vi "Set Input.vi"(8 "error in (no error)":errorcluster caption="에러 입력(에러 없음)", 10 "Input path":T1, 11 "CE RF Switch Box 입력":refnum<class "CE RF Switch Box.lvclass">) -> (0 "error out":errorcluster caption="에러 출력", 3 "CE RF Switch Box 출력":refnum<class "CE RF Switch Box.lvclass">)   [LabVIEW 2023, in "RF Switch Box.lvlib" / "CE RF Switch Box.lvclass"]
uses:
  CE RF Switch Box.lvclass
  Type Definition/Input path.ctl
  CE RF Switch Box.lvclass/CE RF Switch Box.ctl
  RF Switch Box.lvlib
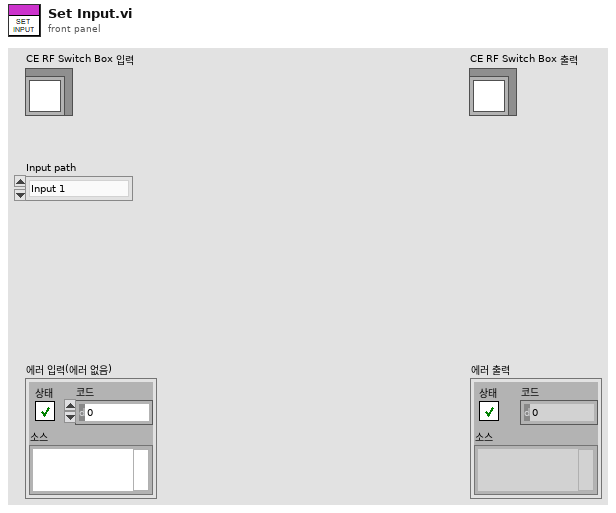
[diagram p1: front panel]
types:
  T1 = typedef "RF Switch Box.lvlib/Input path.ctl" = enum16{"Input 1", "Input 2", "Input 3"}
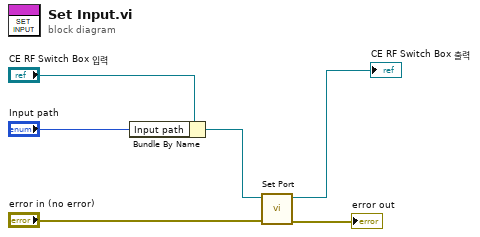
[diagram p0: block diagram]
diagram:
  n1 = Bundle By Name(cluster="CE RF Switch Box 입력", "Input path"="Input path") -> (w4:refnum<class "CE RF Switch Box.lvclass">)
  n2 = call "Set Port.vi"("error in (no error)"="error in (no error)", "CE RF Switch Box 입력"=w4) -> ("error out"=→"error out":errorcluster, "CE RF Switch Box 출력"=→"CE RF Switch Box 출력":refnum<class "CE RF Switch Box.lvclass">)  [unwired: 8 in]
